vi "BUILD_read vip token.vi"(10 "regular expression":string, 11 "data":string) -> (2 "remaining string":string, 3 "trimmed string":string)   [LabVIEW 2010]
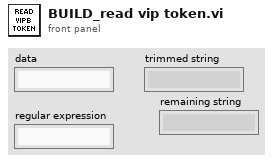
[diagram p1: front panel]
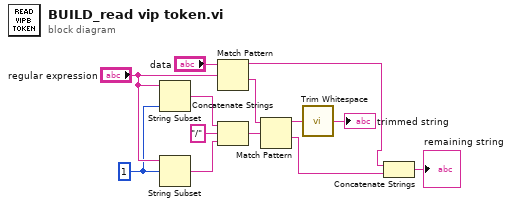
[diagram p0: block diagram]
diagram:
  w4 = 1 ("length (rest)")
  n1 = String Subset(string="regular expression", length (rest)=w4) -> (substring=w5:string)  [unwired: 1 in]
  n2 = String Subset(string="regular expression", offset (0)=w4) -> (substring=w6:string)  [unwired: 1 in]
  n3 = Match Pattern(string="data", regular expression="regular expression") -> (before substring=w2:string, after substring=w12:string)  [unwired: 1 in, 2 out]
  n4 = Concatenate Strings(w5, "/" ("string"), w6) -> (w8:string)
  n5 = Match Pattern(string=w12, regular expression=w8) -> (before substring=w9:string, after substring=w3:string)  [unwired: 1 in, 2 out]
  n6 = call <vilib>:"Trim Whitespace.vi"("string"=w9) -> ("trimmed string"=→"trimmed string":string)  [unwired: 1 in]
  n7 = Concatenate Strings(w2, w3) -> (→"remaining string":string)
